vi "G-Uart-Receive_data.vi"(7 "全读":bool=TRUE, 8 "error in (no error)":errorcluster caption="错误输入（无错误）", 9 "Bytes at Port":u32, 10 "Uart":T1, 11 "G-Uart-Class 输入":refnum<class "G-Uart-Class.lvclass">) -> (0 "error out":errorcluster caption="错误输出", 1 "return count":u32, 2 "read buffer":string, 3 "G-Uart-Class 输出":refnum<class "G-Uart-Class.lvclass">)   [LabVIEW 2025, in "G-Uart-Class.lvclass"]
uses:
  G-Uart-Class.lvclass
  Register-Uart.ctl
  G-Uart-Class.lvclass/G-Uart-Class.ctl
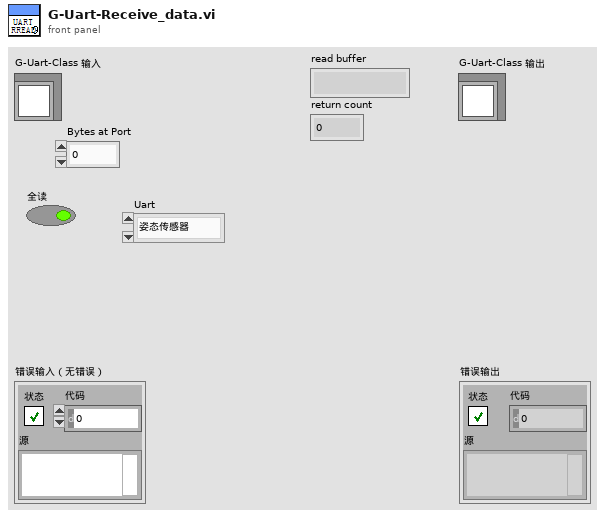
[diagram p1: front panel]
types:
  T1 = typedef "G-Uart-Class.lvclass/Register-Uart.ctl" = enum16{"姿态传感器", "图像跟踪", "观瞄仪器", "电源"}
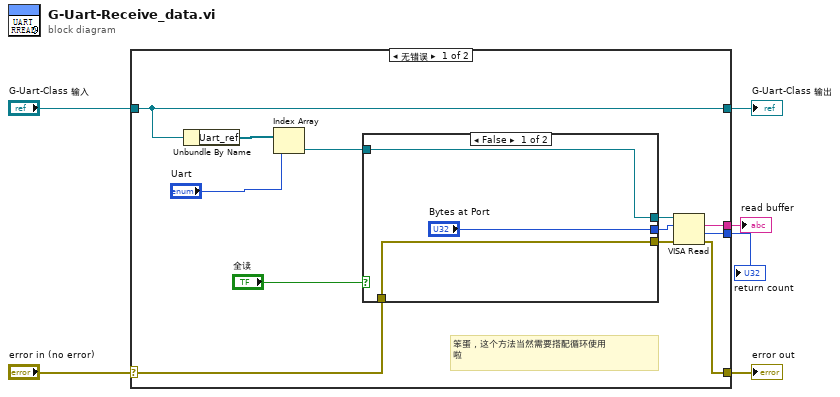
[diagram p0: block diagram]
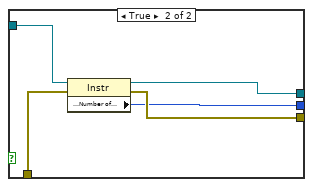
[diagram p2: hidden frame]
diagram:
  n1 = case shown="无错误" "error in (no error)" {
    selector: "error in (no error)" -> [w14 w28]
    tunnel: [w10 w28] -> w5
    tunnel: [w18 w27] -> w3
    tunnel: "G-Uart-Class 输入" -> [w18 w27]
    tunnel: [w9 _] -> w2
    tunnel: [w8 _] -> w1
    frame No Error {
      # "笨蛋，这个方法当然需要搭配循环使用\n啦"
      n2 = Unbundle By Name(w18) -> ("Uart_ref"=w17:refnum<visa-resource-name>[])
      n3 = Index Array(array=w17, index="Uart") -> (element=w15:refnum<visa-resource-name>)
      n4 = case shown="False" "全读" {
        tunnel: w15 -> [w21 w26]
        tunnel: w14 -> [w19 w25]
        tunnel: [w19 w24] -> w13
        tunnel: ["Bytes at Port" w23] -> w12
        tunnel: [w21 w22] -> w11
        frame False {
        }
        frame True {
          n5 = property class="Instr"(reference=w26, error in=w25) -> (reference out=w22:refnum<visa-resource-name>, error out=w24:errorcluster, "Serial Settings:Number of Bytes at Serial Port"=w23:u32)
        }
      }
      n6 = VISA Read(VISA resource name=w11, byte count=w12, error in (no error)=w13) -> (read buffer=w9:string, return count=w8:u32, error out=w10:errorcluster)  [unwired: 1 out]
    }
    frame Error {
    }
  }
  "error out" <- w5
  "G-Uart-Class 输出" <- w3
  "read buffer" <- w2
  "return count" <- w1
